vi "Check_the_User_List.vi"(8 "error in (no error)":errorcluster, 10 "Password":string, 11 "Name":string) -> (0 "error out":errorcluster, 3 "Result":bool)   [LabVIEW 2021]
uses:
  <vilib>/regexp/Match Regular Expression.xnode
panel:
  out "concatenated string":string
  out "standard output":string
  out "standard error":string
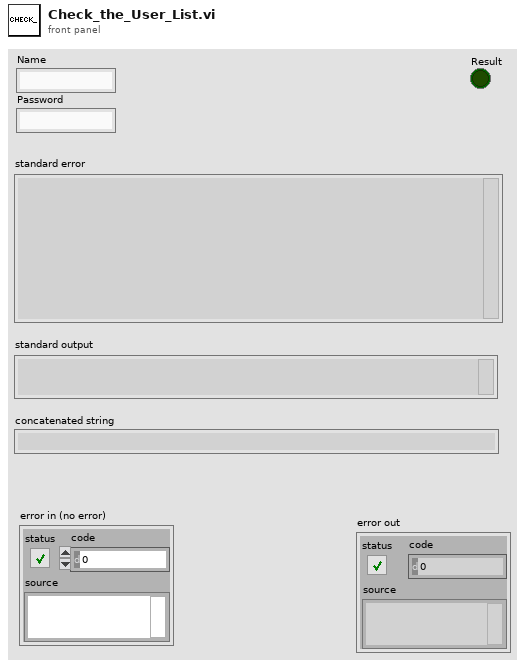
[diagram p1: front panel]
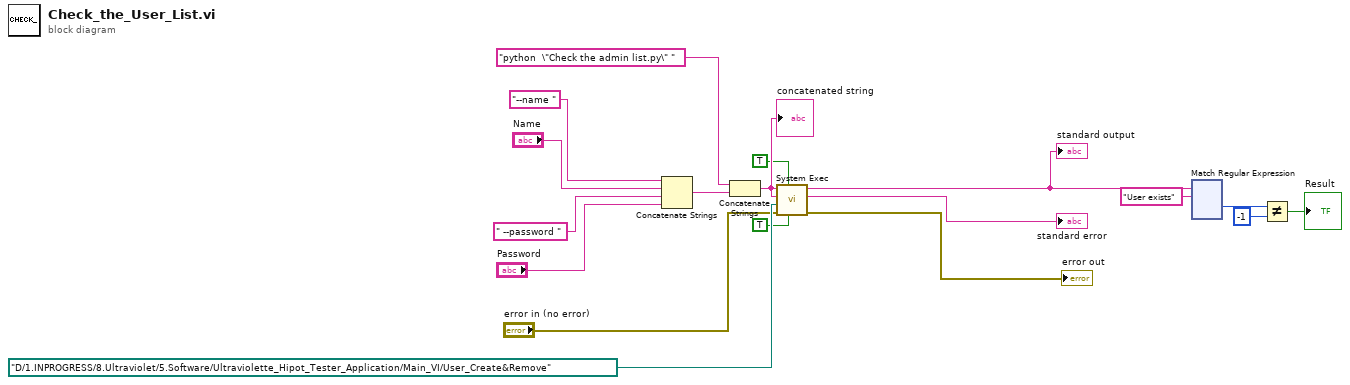
[diagram p0: block diagram]
diagram:
  n1 = Concatenate Strings("--name " ("standard input"), "Name", " --password " ("standard input"), "Password") -> (w8:string)
  n2 = Concatenate Strings("python  \"Check the admin list.py\" " ("command line"), w8) -> (w15:string)
  "concatenated string" <- w15
  n3 = call <vilib>:"System Exec.vi"("run minimized? (F)"=TRUE, "wait until completion? (T)"=TRUE, "error in (no error)"="error in (no error)", "working directory"=path "D:/1.INPROGRESS/8.Ultraviolet/5.Software/Ultraviolette_Hipot_Tester_Application/Main_VI/User_Create&Remove", "standard input"=w15, "command line"=w15) -> ("error out"=→"error out":errorcluster, "standard error"=→"standard error":string, "standard output"=w7:string)  [unwired: 2 in, 1 out]
  "standard output" <- w7
  n4 = xnode "Match Regular Expression"("input string"=w7, "regular expression"="User exists") -> ("offset past match"=w5:i32)  [unwired: 4 in, 4 out]
  n5 = Not Equal?(x=w5, y=-1) -> (x != y?=→"Result":bool)
